vi "Modify Template.vi"(8 "error in":errorcluster, 11 "ILabVIEWFile in":refnum<class "LabVIEW File.lvclass">) -> (0 "error out":errorcluster, 3 "ILabVIEWFile out":refnum<class "LabVIEW File.lvclass">)   [LabVIEW 2026, in "LabVIEW File.lvclass"]
doc: "This method modifies (i.e. adds/removes/replaces elements in the template) to implement the current file."
uses:
  LabVIEW File.lvclass
  LabVIEW File.lvclass/LabVIEW File.ctl
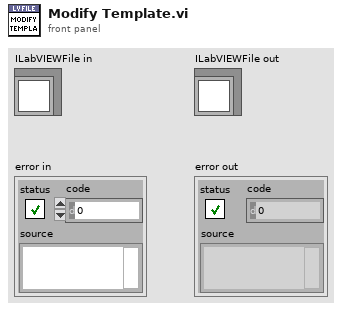
[diagram p1: front panel]
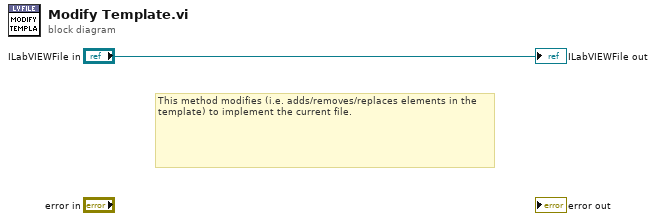
[diagram p0: block diagram]
diagram:
  # "This method modifies (i.e. adds/removes/replaces elements in the template) to implement the current file."
  "ILabVIEWFile out" <- "ILabVIEWFile in"
